vi "ASD Right Read Ratio.vi"(8 "error in":errorcluster caption="エラー入力（エラーなし）", 9 "Right Read MIN":i32=4, 10 "Base Table":T2(array[cluster]) {"Value 3" format="%.2g"}, 11 "Sample Sequence":string="TGTXCT") -> (0 "error out":errorcluster caption="エラー出力", 1 "RR Ratio (%)":dbl format="%.3g", 2 "Right Read MIN out":i32=4, 3 "RR Seq":T1)   [LabVIEW 2018]
panel:
  out "x*y":dbl[](array[numeric])
  in  "Set":bool
  out "x - y":i32
  out "RR Canditate#":i32[](array[numeric])
  out "サイズ":i32
  out "配列 4":i32[](array[numeric])
  out "Cutted Sequence":string
  out "配列 2":string[](array[string])
  out "RR option#":i32
  out "Base Cutted Q#":i32
  out "RRS#":i32
  out "Potential Canditate#":i32[](array[numeric])
  out "all option#":i32
  out "Base Species#":i32
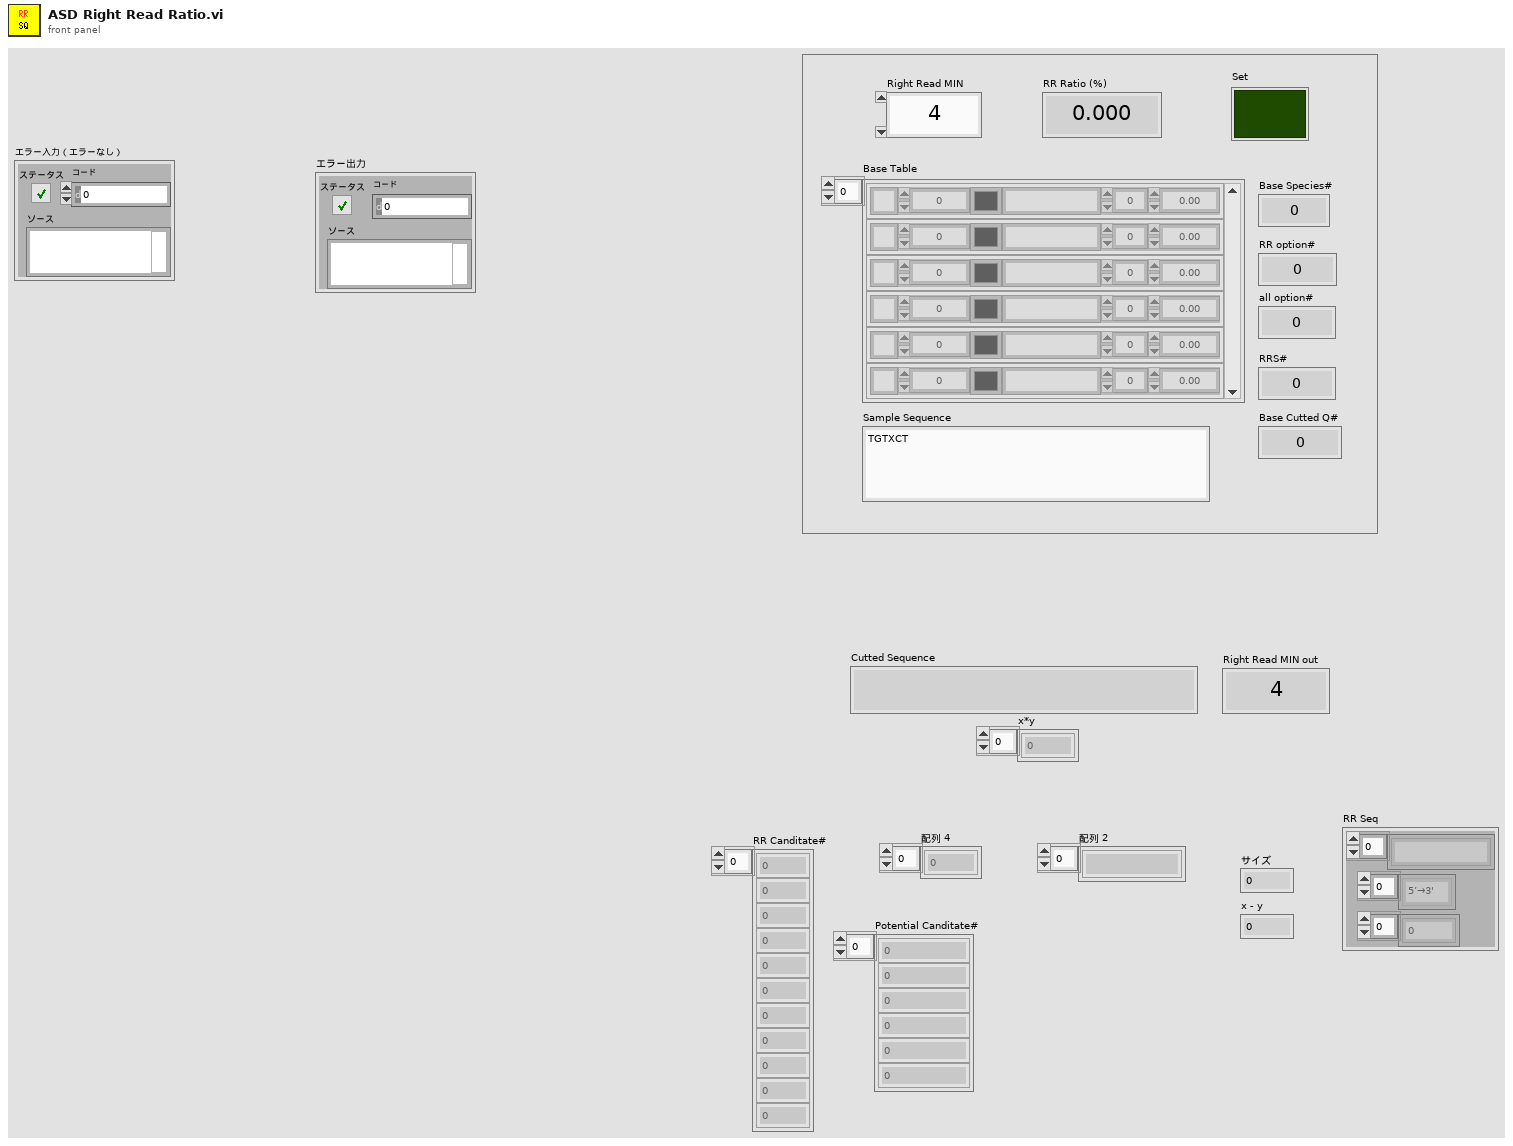
[diagram p1: front panel]
types:
  T1 = cluster{string[], enum16{"5’→3'", "3'→5'"}[], i32[]}
  T2 = cluster{"Name":string, "Value":dbl, "Color":u32, "Name 2":string, "Value 2":dbl, "Value 3":dbl}[]
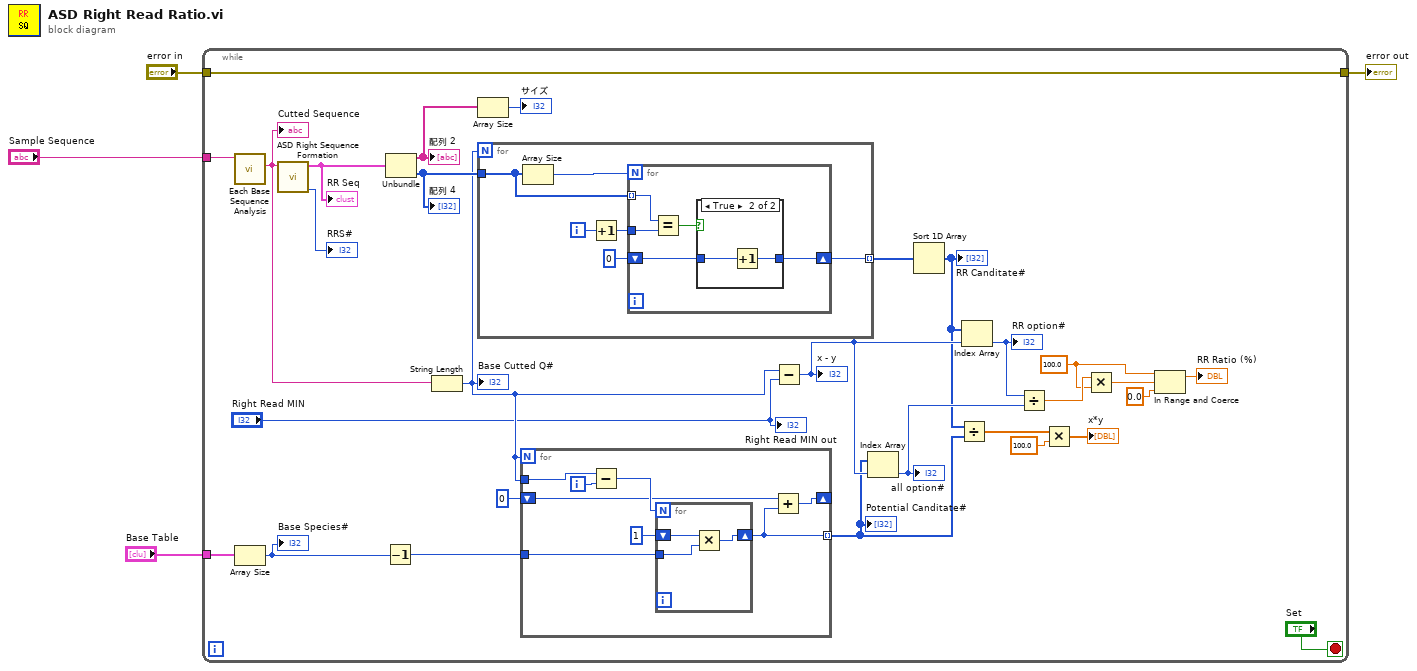
[diagram p0: block diagram]
diagram:
  n1 = while {
    tunnel: "Sample Sequence" -> [w13]
    tunnel: "Base Table" -> [w12]
    tunnel: "error in" -> [w10]
    tunnel: [w10] -> w1
    stop <- "Set" stop-if-true
    w15 = 100.0 ("y")
    n2 = call "Each Base Sequence Analysis.vi"("Sample Sequence"=w13) -> ("Cutted Sequence"=w32:string)  [unwired: 7 in, 3 out]
    "Cutted Sequence" <- w32
    n3 = Array Size(array=w12) -> (size(s)=w33:i32)
    "Base Species#" <- w33
    n4 = call "ASD Right Sequence Formation.vi"("Sample Sequence"=w32) -> ("RRS#"=→"RRS#":i32, "RR Seq"=w26:T1)  [unwired: 9 in]
    "RR Seq" <- w26
    n5 = Decrement(x=w33) -> (x-1=w31:i32)
    n6 = Unbundle(w26) -> (w24:string[], w23:i32[])  [unwired: 1 out]
    "配列 2" <- w24
    "配列 4" <- w23
    n7 = String Length(string=w32) -> (length=w22:i32)
    "Base Cutted Q#" <- w22
    n8 = Array Size(array=w24) -> (size(s)=→"サイズ":i32)
    n9 = for {
      N: w22 -> [_]
      tunnel: w23 -> [w39]
      tunnel: [w36] -> w20 mode=indexing
      i -> [w35]
      n10 = Array Size(array=w39) -> (size(s)=w38:i32)
      n11 = Increment(x=w35) -> (x+1=w34:i32)
      n12 = for {
        N: w38 -> [_]
        tunnel: w39 -> [w44] mode=indexing
        shift-right: [w42] -> w36
        shift-left: 0 -> [w41]
        tunnel: w34 -> [w40]
        n13 = Equal?(x=w44, y=w40) -> (x = y?=w43:bool)
        n14 = case shown="True" w43 {
          tunnel: [w45 w47] -> w42
          tunnel: w41 -> [w45 w46]
          frame False {
          }
          frame True {
            n15 = Increment(x=w46) -> (x+1=w47:i32)
          }
        }
      }
    }
    n16 = for {
      N: w22 -> [_]
      tunnel: w22 -> [w52]
      tunnel: w31 -> [w55]
      shift-right: [w49] -> _
      shift-left: 0 -> [w50]
      tunnel: [w48] -> w8 mode=indexing
      i -> [w51]
      n17 = Subtract(x=w52, y=w51) -> (x-y=w53:i32)
      n18 = for {
        N: w53 -> [_]
        tunnel: w55 -> [w58]
        shift-right: [w57] -> w48
        shift-left: 1 -> [w56]
        n19 = Multiply(x=w56, y=w58) -> (x*y=w57:i32)
      }
      n20 = Add(x=w50, y=w48) -> (x+y=w49:i32)
    }
    "Potential Canditate#" <- w8
    n21 = Subtract(x=w22, y="Right Read MIN") -> (x-y=w18:i32)
    "x - y" <- w18
    n22 = Index Array(array=w8, index=w18) -> (element=w27:i32)
    "all option#" <- w27
    n23 = Sort 1D Array(array=w20) -> (sorted array=w9:i32[])
    "RR Canditate#" <- w9
    n24 = Divide(x=w9, y=w8) -> (x/y=w6:dbl[])
    n25 = Index Array(array=w9, index=w18) -> (element=w21:i32)
    "RR option#" <- w21
    n26 = Divide(x=w21, y=w27) -> (x/y=w28:dbl)
    n27 = Multiply(x=w6, y=100.0) -> (x*y=→"x*y":dbl[])
    n28 = Multiply(x=w28, y=w15) -> (x*y=w17:dbl)
    n29 = In Range and Coerce(upper limit=w15, x=w17, lower limit=0.0 ("下限")) -> (coerced(x)=→"RR Ratio (%)":dbl)  [unwired: 1 out]
    "Right Read MIN out" <- "Right Read MIN"
  }
  "error out" <- w1
